vi "Math Test Suite.vi"() -> ()   [LabVIEW 2020]
doc: "This example demonstrates how to programmatically save the test report to a file."
uses:
  classes/Test Result/Node Results.ctl
  classes/Test Result/Test Node.ctl
  classes/Test Result/Test Registration Data.ctl
  classes/Test Result/Assert Event Data.ctl
  classes/Test Suite/Test Suite.lvclass
  classes/Test Result/Test Result.lvclass
panel:
  out "Legacy Test Results":T1[](array[typedef])
  in  "error in (no error)":errorcluster
  out "error out":errorcluster
  # "See block diagram"
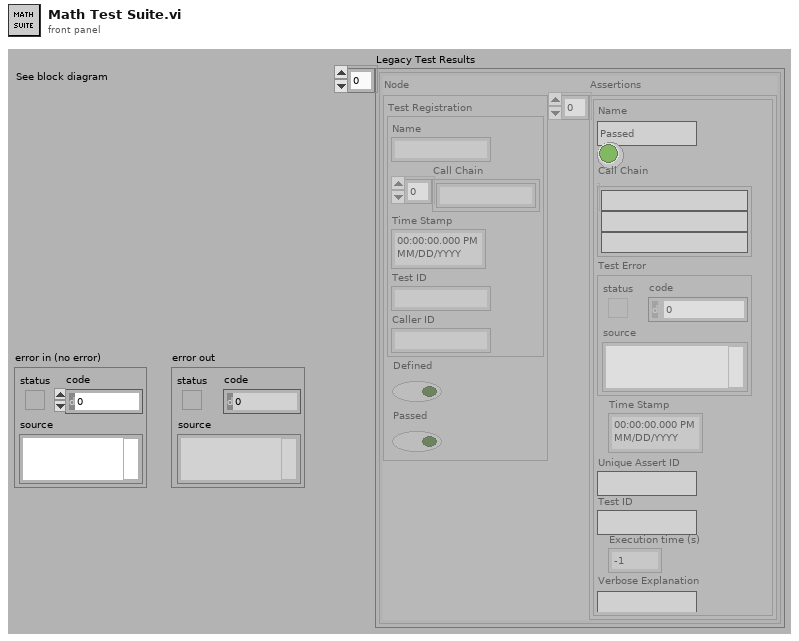
[diagram p1: front panel]
types:
  T1 = typedef "Caraya.lvlib/Test Result.lvclass/Node Results.ctl" = cluster{"Node":T2, "Assertions":T4[]}
  T2 = typedef "Caraya.lvlib/Test Result.lvclass/Test Node.ctl" = cluster{"Test Registration":T3, "Defined":bool, "Passed":bool}
  T3 = typedef "Caraya.lvlib/Test Result.lvclass/Test Registration Data.ctl" = cluster{"Name":string, "Call Chain":string[], "Time Stamp":timestamp, "Test ID":string, "Caller ID":string}
  T4 = typedef "Caraya.lvlib/Test Result.lvclass/Assert Event Data.ctl" = cluster{"Name":string, "Passed":bool, "Call Chain":string[], "Test Error":errorcluster, "Time Stamp":timestamp, "Unique Assert ID":string, "Test ID":string, "Execution time (s)":dbl, "Verbose Explanation":string}
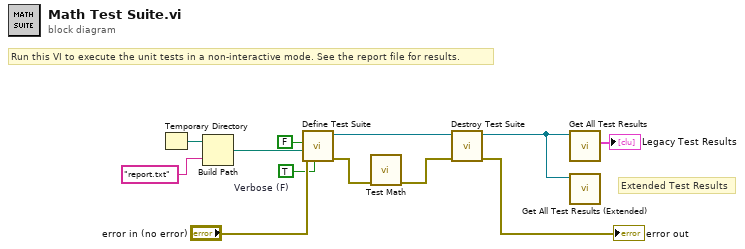
[diagram p0: block diagram]
diagram:
  w5 = TRUE  # Verbose (F)
  # "Extended Test Results"
  # "Run this VI to execute the unit tests in a non-interactive mode. See the report file for results."
  n1 = Temporary Directory() -> (w9:path)
  n2 = Build Path(base path=w9, name or relative path="report.txt") -> (appended path=w7:path)
  n3 = call "Define Test Suite.vi"("Verbose (F)"=w5, "error in (no error)"="error in (no error)", "Report Path"=w7, "Interactive"=FALSE) -> ("error out"=w3:errorcluster, "Test Suite"=w4:refnum<class "Test Suite.lvclass">)  [unwired: 5 in, 1 out]
  n4 = call "Test Math.vi"("error in (no error)"=w3) -> ("error out"=w12:errorcluster)  [unwired: 10 in]
  n5 = call-dynamic "Destroy Test Suite.vi"("error in (no error)"=w12, "Test Suite in"=w4) -> ("error out"=→"error out":errorcluster, "Test Suite Results"=w1:refnum<class "Test Result.lvclass">)  [unwired: 8 in]
  n6 = call "Get All Test Results.vi"("Test Result in"=w1) -> ("Test Results"=→"Legacy Test Results":T1[])  [unwired: 8 in, 2 out]
  n7 = call "Get All Test Results (Extended).vi"("Test Result in"=w1) -> ()  [unwired: 8 in, 3 out]
